vi "Module Loop.vi"(8 "error in (no error)":errorcluster, 11 "GUI Manager Module in":refnum<class "GUI Manager Module.lvclass">) -> (0 "error out":errorcluster, 3 "GUI Manager Module out":refnum<class "GUI Manager Module.lvclass">)   [LabVIEW 2020, in "VolatusGUI.lvlib" / "GUI Manager Module.lvclass"]
uses:
  GUI Manager Module.lvclass
  C:/dev/lv20CE/relink/lv-volatus/Volatus/Module/Module.lvclass
  GUI Entry.ctl
  Volatus/Module/Module.lvclass/Module.ctl
  Volatus/MessageQ/MessageQ.lvclass/MessageQ.ctl
  lv-promises/Promises/Variant/Variant.lvclass/Variant.ctl
  Volatus/Module/Module.lvclass
  Volatus/Event Reporter Identity/Event Reporter Identity.lvclass
  C:/dev/lv20CE/relink/lv-volatus/Volatus/Identity/Identity.lvclass
  Volatus/Events Summary Value/Events Summary Value.lvclass
  GUI Registration.ctl
  Volatus/MessageQ/MessageQ.lvclass
  GUI Info.ctl
  GUI Manager Module.lvclass/GUI Manager Module.ctl
  Unregister GUI.ctl
  System Status Module/System Status Module.lvclass
  VolatusConfig/VolatusConfigElement/VolatusConfigElement.lvclass
  Volatus/Roles API/Roles API.lvclass
  Visibility Data.ctl
  Position Data.ctl
  <vilib>/Utility/miscctls.llb/LVRectTypeDef.ctl
  Event Viewer Identity/Event Viewer Identity.lvclass
  Volatus/Roles API/Roles API.lvclass/Roles API.ctl
  Volatus/Module Identity/Module Identity.lvclass/Module Identity.ctl
  782c3c59-6500-4745-abed-eb8793f80122.vi
  Volatus/Module Identity/Module Identity.lvclass
  <vilib>/Utility/error.llb/Error Cluster From Error Code.vi
  lv-promises/Promises/Variant/Variant.lvclass
  lv-promises/Promises/Promise/Promise.lvclass
  VolatusGUI.lvlib
  GUIStateValue/GUIStateValue.lvclass
  Volatus/VolatusAPI/VolatusAPI.lvclass
  Volatus/Volatus.lvlib
  GUI Helper/GUI Helper.lvclass
panel:
  out "Cmd Status":cluster{"Net Color":u32, "Net Status":string}
  in  "Event Log":bool
  out "Warnings":i32
  out "Errors":i32
  in  "Role Status":T1
  in  "GUIs":T2[](array[typedef])
  # "WARN"
  # "ERR"
  # "Commands"
  # "Role"
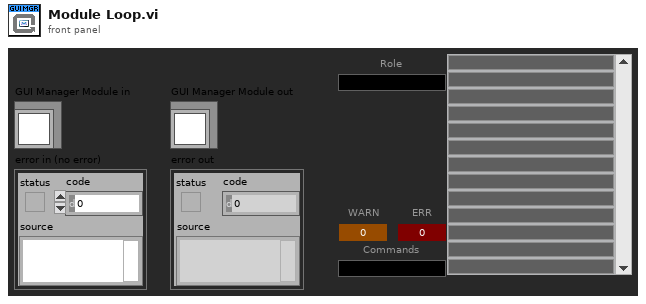
[diagram p1: front panel]
types:
  T1 = cluster{"Color":u32, "Role":string, "Select Role":bool}
  T2 = typedef "VolatusGUI.lvlib/GUI Manager Module.lvclass/GUI Entry.ctl" = cluster{"Name Color":u32, "Name":string, "Show GUI":bool, "ID":string}
  T3 = cluster{"Name Color":bool, "Name":bool, "Show GUI":bool, "ID":bool}[]
  T4 = enum32{"Invalid", "Standard", "Closed", "Hidden", "Minimized", "Maximized"}
  T5 = typedef "VolatusGUI.lvlib/GUI Registration.ctl" = cluster{"ID":string, "GUI Helper":refnum<class "MessageQ.lvclass">, "Module":refnum<class "MessageQ.lvclass">, "Info":T6, "Open":bool}
  T6 = typedef "VolatusGUI.lvlib/GUI Info.ctl" = cluster{"Color":u32, "Name":string}
  T7 = typedef "VolatusGUI.lvlib/Unregister GUI.ctl" = cluster{"Name":string}
  T8 = typedef "VolatusGUI.lvlib/Visibility Data.ctl" = cluster{"GUI ID":string, "Visible":bool}
  T9 = typedef "VolatusGUI.lvlib/Position Data.ctl" = cluster{"GUI ID":string, "Bounds":T10}
  T10 = typedef "LVRectTypeDef.ctl" = cluster{"Left":i16, "Top":i16, "Right":i16, "Bottom":i16}
  T11 = typedef "Volatus.lvlib/Events Summary.ctl" = cluster{"# Debug":i32, "# Info":i32, "# Warning":i32, "# Error":i32}
  T12 = typedef "VolatusGUI.lvlib/GUI State.ctl" = cluster{"GUI ID":string, "Visible":bool, "Visibility Set":bool, "Bounds":T10, "Bounds Set":bool}
  T13 = typedef "VolatusGUI.lvlib/GUI Manager Module.lvclass/Plugin Info.ctl" = cluster{"Path":path, "Module ID":string, "Filename":string}
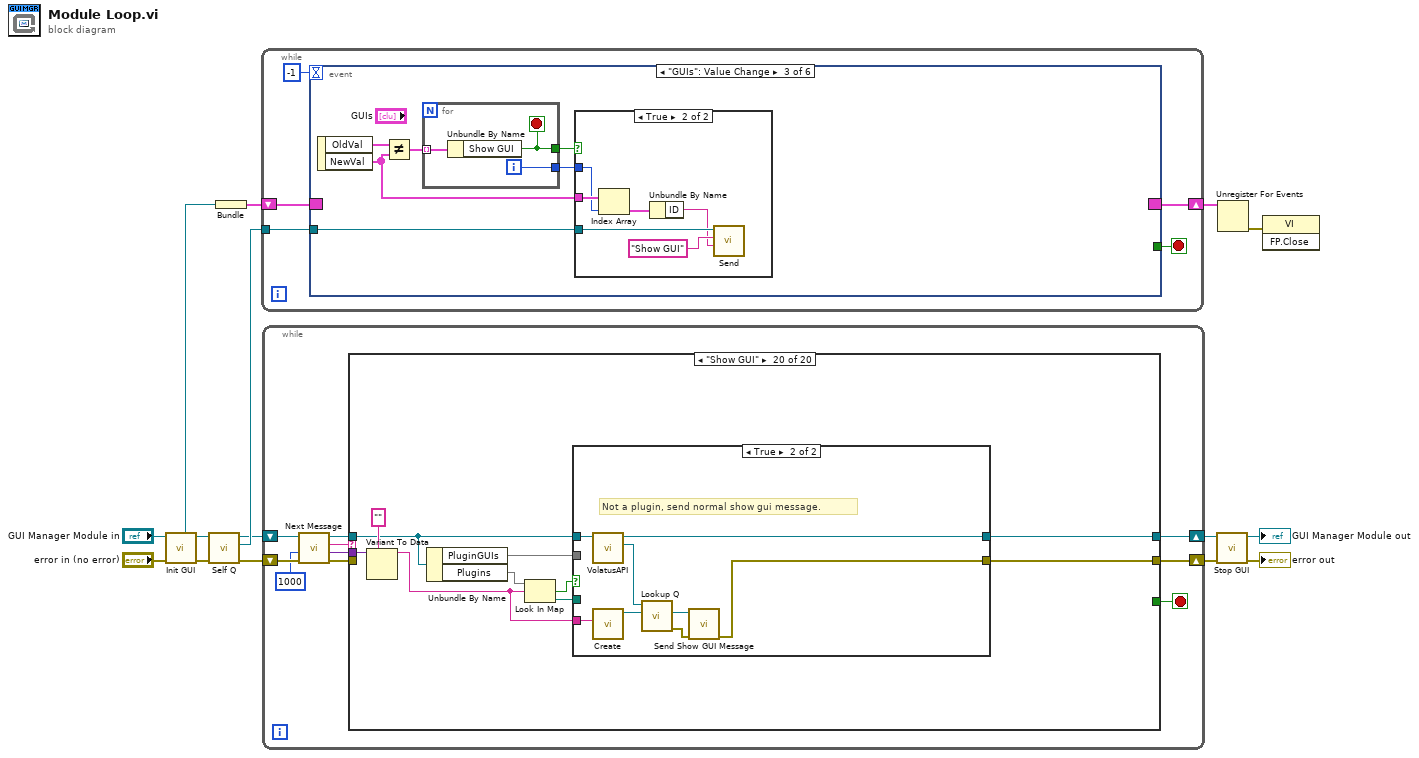
[diagram p0: block diagram]
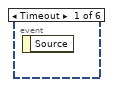
[diagram p2: hidden frame]
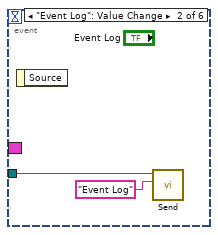
[diagram p3: hidden frame]
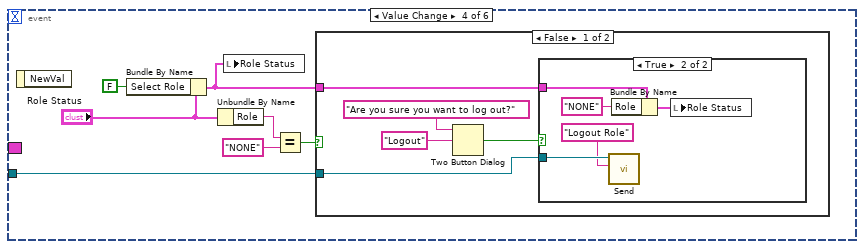
[diagram p5: hidden frame]
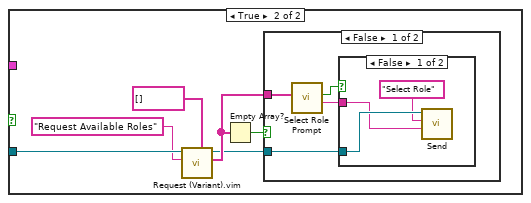
[diagram p7: hidden frame]
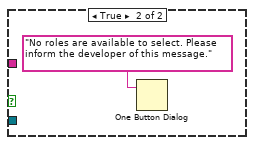
[diagram p9: hidden frame]
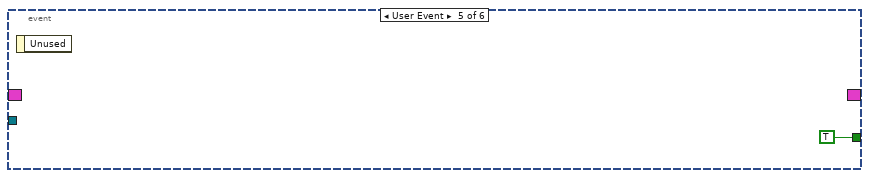
[diagram p10: hidden frame]
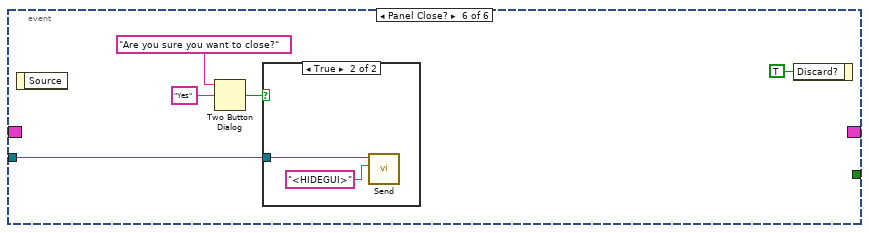
[diagram p11: hidden frame]
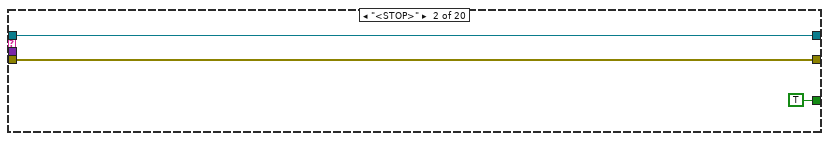
[diagram p14: hidden frame]
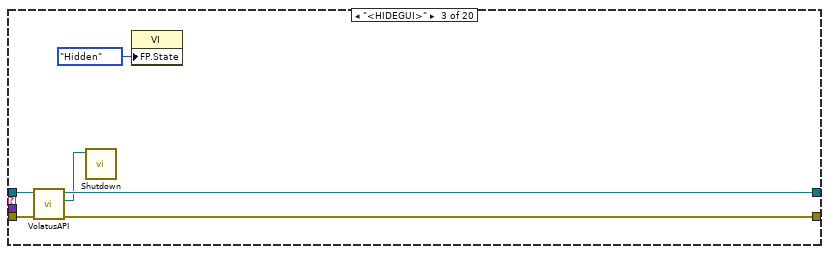
[diagram p15: hidden frame]
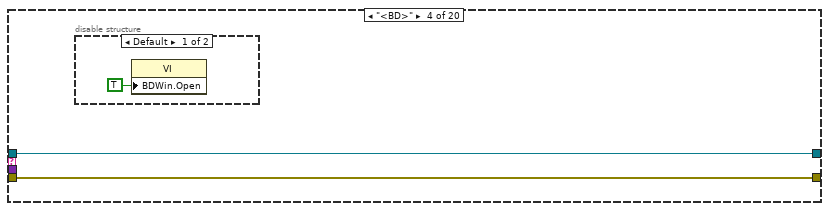
[diagram p16: hidden frame]
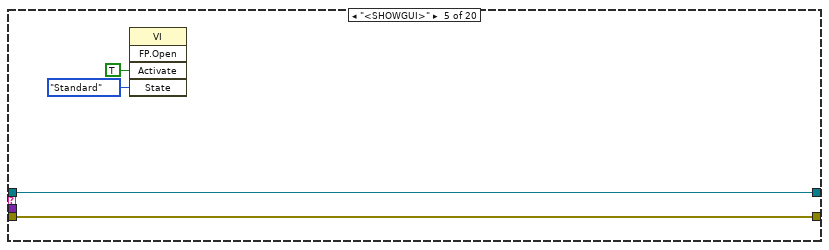
[diagram p18: hidden frame]
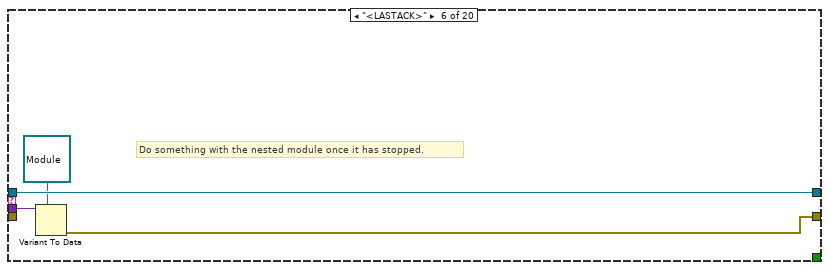
[diagram p19: hidden frame]
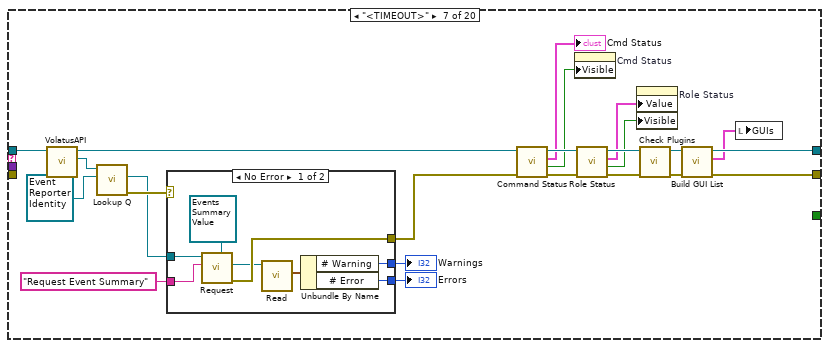
[diagram p20: hidden frame]
diagram:
  n1 = call "Init GUI.vi"("Module in"="GUI Manager Module in") -> ("Module out"=w9:refnum<class "GUI Manager Module.lvclass">, "Event Reg"=w12:refnum<event-registration>)  [unwired: 9 in]
  n2 = call "Self Q.vi"("Module in"=w9) -> ("Self Q"=w8:refnum<class "MessageQ.lvclass">, "Module out"=w7:refnum<class "GUI Manager Module.lvclass">)  [unwired: 9 in]
  n3 = Bundle("Event Reg"=w12) -> (w10:cluster{"Event Reg":refnum<event-registration>})  [unwired: 1 in]
  n4 = while {
    tunnel: w8 -> [w18]
    shift-right: [w16] -> w11
    shift-left: w10 -> [w17]
    stop <- w15 stop-if-true
    n5 = event shown="[2] \"GUIs\": Value Change" {
      selector: w17 -> [_ _ _ _ _ _]
      dyn-events: [_ _ _ _ _ _] -> w16
      timeout: -1 -> [_ _ _ _ _ _]
      tunnel: w18 -> [_ w20 w21 w42 _ w68]
      tunnel: [_ _ _ _ TRUE _] -> w15
      event Timeout {
        n6 = event-data() -> ()  [unwired: 1 in, 1 out]
      }
      event "Event Log": Value Change {
        n7 = event-data() -> ()  [unwired: 1 in, 1 out]
        n8 = call "Send.vi"("ID"="Event Log", "MessageQ in"=w20) -> ()  [unwired: 8 in, 2 out]
      }
      event "GUIs": Value Change {
        n9 = event-data() -> ("OldVal"=w26:T2[], "NewVal"=w22:T2[])  [unwired: 1 in]
        n10 = Not Equal?(x=w26, y=w22) -> (x != y?=w25:T3)
        n11 = for {
          tunnel: w25 -> [w35] mode=indexing
          tunnel: [w34] -> w24
          tunnel: [w33] -> w23
          i -> [w33]
          stop <- w34 stop-if-true
          n12 = Unbundle By Name(w35) -> ("Show GUI"=w34:bool)
        }
        n13 = case shown="True" w24 {
          tunnel: w23 -> [_ w31]
          tunnel: w22 -> [_ w32]
          tunnel: w21 -> [_ w29]
          frame False {
          }
          frame True {
            n14 = Index Array(array=w32, index=w31) -> (element=w30:T2)
            n15 = Unbundle By Name(w30) -> ("ID"=w27:string)
            n16 = call "Send.vi"("Data"=w27, "ID"="Show GUI", "MessageQ in"=w29) -> ()  [unwired: 7 in, 2 out]
          }
        }
      }
      event "Role Status.Select Role": Value Change {
        n17 = event-data() -> ()  [unwired: 1 in, 1 out]
        n18 = Bundle By Name(cluster="Role Status", "Select Role"=FALSE) -> (w36:T1)
        n19 = Unbundle By Name("Role Status") -> ("Role"=w41:string)
        n20 = local write "Role Status"(w36) -> ()
        n21 = Equal?(x=w41, y="NONE") -> (x = y?=w39:bool)
        n22 = case shown="False" w39 {
          tunnel: w42 -> [w47 w58]
          tunnel: w36 -> [w43 _]
          frame False {
            n23 = Two Button Dialog(message="Are you sure you want to log out?", 2:"Logout" ("T button name (\"OK\")")) -> (T button?=w44:bool)  [unwired: 1 in]
            n24 = case shown="True" w44 {
              tunnel: w47 -> [_ w52]
              tunnel: w43 -> [_ w50]
              frame False {
              }
              frame True {
                n25 = call "Send.vi"("ID"="Logout Role", "MessageQ in"=w52) -> ()  [unwired: 8 in, 2 out]
                n26 = Bundle By Name(cluster=w50, "Role"="NONE") -> (w48:T1)
                n27 = local write "Role Status"(w48) -> ()
              }
            }
          }
          frame True {
            n28 = call "Request (Variant).vim"("Type"=string[] [], "ID"="Request Available Roles", "MessageQ in"=w58) -> ("Value"=w54:string[], "MessageQ out"=w53:refnum<class "MessageQ.lvclass">)  [unwired: 6 in, 1 out]
            n29 = Empty Array?(array=w54) -> (empty?=w55:bool)
            n30 = case shown="False" w55 {
              tunnel: w54 -> [w62 _]
              tunnel: w53 -> [w61 _]
              frame False {
                n31 = call "Select Role Prompt.vi"("Available Roles"=w62) -> ("Selected Role"=w59:string, "Cancelled"=w60:bool)  [unwired: 9 in]
                n32 = case shown="False" w60 {
                  tunnel: w61 -> [w65 _]
                  tunnel: w59 -> [w64 _]
                  frame False {
                    n33 = call "Send.vi"("Data"=w64, "ID"="Select Role", "MessageQ in"=w65) -> ()  [unwired: 7 in, 2 out]
                  }
                  frame True {
                  }
                }
              }
              frame True {
                n34 = One Button Dialog(message="No roles are available to select. Please inform the developer of this message.") -> ()  [unwired: 1 in, 1 out]
              }
            }
          }
        }
      }
      event User Event {
        n35 = event-data() -> ()  [unwired: 1 in, 1 out]
      }
      event Panel Close? {
        n36 = event-data() -> ()  [unwired: 1 in, 1 out]
        n37 = Two Button Dialog(message="Are you sure you want to close?", 2:"Yes" ("T button name (\"OK\")")) -> (T button?=w69:bool)  [unwired: 1 in]
        n38 = case shown="True" w69 {
          tunnel: w68 -> [_ w73]
          frame False {
          }
          frame True {
            n39 = call "Send.vi"("ID"="<HIDEGUI>", "MessageQ in"=w73) -> ()  [unwired: 8 in, 2 out]
          }
        }
        n40 = event-data("Discard?"=TRUE) -> ()  [unwired: 1 in, 1 out]
      }
    }
  }
  n41 = while {
    shift-right: [w79] -> w4
    shift-left: w7 -> [w84]
    shift-right: [w78] -> w3
    shift-left: "error in (no error)" -> [w83]
    stop <- w77 stop-if-true
    n42 = call "Next Message.vi"("error in (no error)"=w83, "Timeout ms (-1)"=1000, "Module in"=w84) -> ("error out"=w82:errorcluster, "Data"=w76:variant, "ID"=w81:string, "Module out"=w80:refnum<class "GUI Manager Module.lvclass">)  [unwired: 5 in]
    n43 = case shown="\"Show GUI\"" w81 {
      tunnel: w82 -> [w85 w88 w93 w95 w100 _ _ _ _ w167 w186 _ w201 _ _ _ _ _ _ _]
      tunnel: w80 -> [w86 w89 w94 w96 w101 w105 w112 w141 w157 w165 w183 w194 w197 w215 w229 w240 w246 w251 w256 w262]
      tunnel: [w86 w89 w91 w96 w101 w105 w121 w137 w154 w164 w173 w191 w195 w212 w223 w239 w246 w251 w256 w264] -> w79
      tunnel: [w85 w88 w93 w95 w100 w102 w123 w138 w155 w166 w175 w189 w196 w209 w233 w234 w241 w247 w254 w263] -> w78
      tunnel: [_ TRUE _ _ _ _ _ _ _ _ _ _ _ _ _ _ _ _ _ _] -> w77
      tunnel: w76 -> [_ _ _ _ _ w104 _ w143 w159 _ _ w193 w202 w214 w232 _ w244 w253 _ w266]
      frame "<CLOSE>" {
      }
      frame "<STOP>" {
      }
      frame "<HIDEGUI>" {
        n44 = call "VolatusAPI.vi"("Module in"=w94) -> ("VolatusAPI"=w90:refnum<class "VolatusAPI.lvclass">, "Module out"=w91:refnum<class "GUI Manager Module.lvclass">)  [unwired: 9 in]
        n45 = call "Shutdown.vi"("VolatusAPI in"=w90) -> ()  [unwired: 9 in, 2 out]
        n46 = property class="VI"("FP.State"=T4."Hidden" ("Front Panel Window:State")) -> ()  [unwired: 2 in, 2 out]
      }
      frame "<BD>" {
        n47 = disable-structure shown="Default" {
          frame condition #0 (active) {
            n48 = property class="VI"("BDWin.Open"=TRUE ("Block Diagram Window:Open")) -> ()  [unwired: 2 in, 2 out]
          }
          frame condition #1 {
          }
        }
      }
      frame "<SHOWGUI>" {
        n49 = invoke class="VI" method="FP.Open"("Activate"=TRUE ("Activate?"), "State"=T4."Standard") -> ()  [unwired: 3 in, 5 out]
      }
      frame "<LASTACK>" {
        # "Do something with the nested module once it has stopped."
        n50 = Variant To Data(type=refnum<class "Module.lvclass"> refnum ("Volatus:Module"), Variant=w104) -> (error out=w102:errorcluster)  [unwired: 1 in, 1 out]
      }
      frame "<TIMEOUT>" {
        n51 = call "VolatusAPI.vi"("Module in"=w112) -> ("VolatusAPI"=w113:refnum<class "VolatusAPI.lvclass">, "Module out"=w110:refnum<class "GUI Manager Module.lvclass">)  [unwired: 9 in]
        n52 = call "Lookup Q.vi"("Identity"=refnum<class "Event Reporter Identity.lvclass"> refnum ("Volatus:Event Reporter Identity.lvclass"), "VolatusAPI in"=w113) -> ("error out"=w128:errorcluster, "MessageQ"=w111:refnum<class "MessageQ.lvclass">)  [unwired: 7 in, 1 out]
        n53 = case shown="No Error" w128 {
          tunnel: "Request Event Summary" ("ID") -> [w135 _]
          tunnel: [w131 _] -> w126
          tunnel: [w130 _] -> w125
          tunnel: w111 -> [w129 _]
          tunnel: [w136 _] -> w109
          frame No Error {
            n54 = call "Request.vi"("Response Type (None)"=refnum<class "Events Summary Value.lvclass"> refnum ("Volatus:Events Summary Value.lvclass"), "ID"=w135, "MessageQ in"=w129) -> ("error out"=w136:errorcluster, "Response"=w133:refnum<class "Events Summary Value.lvclass">)  [unwired: 6 in, 1 out]
            n55 = call "Read.vi"("Events Summary Value in"=w133) -> ("Events Summary"=w132:T11)  [unwired: 10 in]
            n56 = Unbundle By Name(w132) -> ("# Warning"=w131:i32, "# Error"=w130:i32)
          }
          frame Error {
          }
        }
        "Errors" <- w125
        "Warnings" <- w126
        n57 = call "Command Status.vi"("error in (no error)"=w109, "GUI Manager Module in"=w110) -> ("error out"=w108:errorcluster, "Cmd Active"=w117:bool, "Cmd Status"=→"Cmd Status":cluster{u32, string}, "GUI Manager Module out"=w119:refnum<class "GUI Manager Module.lvclass">)  [unwired: 6 in]
        n58 = property on="Cmd Status" class="Clust (strict)"("Visible"=w117) -> ()  [unwired: 2 in, 2 out]
        n59 = call "Role Status.vi"("error in (no error)"=w108, "GUI Manager Module in"=w119) -> ("error out"=w107:errorcluster, "Roles Active"=w114:bool, "Role Status"=w115:T1, "GUI Manager Module out"=w116:refnum<class "GUI Manager Module.lvclass">)  [unwired: 6 in]
        n60 = property on="Role Status" class="Clust (strict)"("Value"=w115, "Visible"=w114) -> ()  [unwired: 2 in, 2 out]
        n61 = call "Check Plugins.vi"("error in (no error)"=w107, "GUI Manager Module in"=w116) -> ("error out"=w124:errorcluster, "GUI Manager Module out"=w122:refnum<class "GUI Manager Module.lvclass">)  [unwired: 8 in]
        n62 = call "Build GUI List.vi"("error in (no error)"=w124, "GUI Manager Module in"=w122) -> ("error out"=w123:errorcluster, "GUIs"=w120:T2[], "GUI Manager Module out"=w121:refnum<class "GUI Manager Module.lvclass">)  [unwired: 7 in]
        n63 = local write "GUIs"(w120) -> ()
      }
      frame "Register GUI" {
        n64 = Variant To Data(type=T5 {"ID"="", "GUI Helper"=refnum, "Module"=refnum, "Info"={"Color"=0, "Name"=""}, "Open"=FALSE} ("GUI Registration"), Variant=w143) -> (data=w140:T5, error out=w139:errorcluster)  [unwired: 1 in]
        n65 = case shown="No Error" w139 {
          selector: w139 -> [_ w153]
          tunnel: w141 -> [w147 w152]
          tunnel: w140 -> [w145 _]
          tunnel: [_ w153] -> w138
          tunnel: [w144 w152] -> w137
          frame No Error {
            n66 = Unbundle By Name(w145) -> ("ID"=w146:string)
            n67 = in-place {
              in-place-border: w146 -> [w150]
              in-place-border: w145 -> [w149]
              n68 = in-place-cluster #1(w147) -> ("GUIs"=w151:map{string, T5})
              n69 = Insert Into Map(map in=w151, key=w150, value=w149) -> (map out=w148:map{string, T5})  [unwired: 2 out]
              n70 = in-place-cluster #1("GUIs"=w148) -> (w144:refnum<class "GUI Manager Module.lvclass">)
            }
          }
          frame Error {
          }
        }
      }
      frame "Unregister GUI" {
        n71 = Variant To Data(type=T7 {"Name"=""} ("Unregister GUI"), Variant=w159) -> (data=w156:T7, error out=w155:errorcluster)  [unwired: 1 in]
        n72 = in-place {
          in-place-border: w156 -> [w163]
          n73 = in-place-cluster #2(w157) -> ("GUIs"=w162:map{string, T5})
          n74 = Unbundle By Name(w163) -> ("Name"=w161:string)
          n75 = Remove From Map(10:w161, 11:w162) -> (3:w160:map{string, T5})  [unwired: 2 out]
          n76 = in-place-cluster #2("GUIs"=w160) -> (w154:refnum<class "GUI Manager Module.lvclass">)
        }
      }
      frame Default {
        n77 = call "Report Unhandled Message ID.vi"("error in (no error)"=w167, "Module in"=w165) -> ("error out"=w166:errorcluster, "Module out"=w164:refnum<class "GUI Manager Module.lvclass">)  [unwired: 8 in]
      }
      frame "Initialize" {
        n78 = control-ref of="This VI"() -> (w185:refnum<vi>)
        n79 = call "Send Show GUI Message.vi"("error in (no error)"=w186, "Module in"=w183) -> ("error out"=w184:errorcluster, "Module out"=w182:refnum<class "GUI Manager Module.lvclass">)  [unwired: 8 in]
        n80 = call "Launch as Nested.vi"("Register (T)"=FALSE, "error in (no error)"=w184, "GUI"=w185, "Parent in"=w182) -> ("error out"=w169:errorcluster, "Parent"=w170:refnum<class "GUI Manager Module.lvclass">)  [unwired: 5 in, 1 out]
        n81 = call "Subscribe to Roles.vi"("error in (no error)"=w169, "Module in"=w170) -> ("error out"=w187:errorcluster, "Module out"=w168:refnum<class "GUI Manager Module.lvclass">)  [unwired: 8 in]
        n82 = Unbundle By Name(w168) -> ("Title"=w177:string)
        n83 = Empty String/Path?(string/path=w177) -> (empty?=w178:bool)
        n84 = case shown="False" w178 {
          tunnel: w177 -> [w188 _]
          frame False {
            n85 = property class="VI"("Front Panel.Title"=w188) -> ()  [unwired: 2 in, 2 out]
          }
          frame True {
          }
        }
        n86 = call "Check Plugins.vi"("error in (no error)"=w187, "GUI Manager Module in"=w168) -> ("error out"=w181:errorcluster, "GUI Manager Module out"=w179:refnum<class "GUI Manager Module.lvclass">)  [unwired: 8 in]
        n87 = call "Check Plugin Visibility.vi"("error in (no error)"=w181, "GUI Manager Module in"=w179) -> ("error out"=w180:errorcluster, "GUI Manager Module out"=w174:refnum<class "GUI Manager Module.lvclass">)  [unwired: 8 in]
        n88 = call "Launch Nested.vi"("error in (no error)"=w180, "Config Element"=refnum<class "VolatusConfigElement.lvclass"> refnum, "Nested Module"=refnum<class "System Status Module.lvclass"> refnum ("VolatusGUI:System Status Module.lvclass"), "Parent in"=w174) -> ("error out"=w175:errorcluster, "Parent out"=w173:refnum<class "GUI Manager Module.lvclass">)  [unwired: 5 in, 1 out]
      }
      frame "Update Roles" {
        n89 = Variant To Data(type=refnum<class "Roles API.lvclass"> refnum ("Volatus:Roles API.lvclass"), Variant=w193) -> (data=w190:refnum<class "Roles API.lvclass">, error out=w189:errorcluster)  [unwired: 1 in]
        n90 = Bundle By Name(cluster=w194, "Roles"=w190) -> (w191:refnum<class "GUI Manager Module.lvclass">)
      }
      frame "Update Visibility" {
        n91 = Variant To Data(error in=w201, type=T8 {"GUI ID"="", "Visible"=FALSE} ("Visibility Data"), Variant=w202) -> (data=w199:T8, error out=w198:errorcluster)
        n92 = case shown="No Error" w198 {
          selector: w198 -> [_ w207]
          tunnel: w199 -> [w205 _]
          tunnel: w197 -> [w206 w208]
          tunnel: [w204 w207] -> w196
          tunnel: [w203 w208] -> w195
          frame No Error {
            n93 = call "Store Visibility.vi"("Visibility Data"=w205, "GUI Manager Module in"=w206) -> ("error out"=w204:errorcluster, "GUI Manager Module out"=w203:refnum<class "GUI Manager Module.lvclass">)  [unwired: 8 in]
          }
          frame Error {
          }
        }
      }
      frame "Update Position" {
        n94 = Variant To Data(type=T9 {"GUI ID"="", "Bounds"={"Left"=0, "Top"=0, "Right"=0, "Bottom"=0}} ("Position Message"), Variant=w214) -> (data=w211:T9, error out=w210:errorcluster)  [unwired: 1 in]
        n95 = case shown="No Error" w210 {
          selector: w210 -> [w217 w222]
          tunnel: w215 -> [w220 w221]
          tunnel: [w219 w221] -> w212
          tunnel: w211 -> [w218 _]
          tunnel: [w216 w222] -> w209
          frame No Error {
            n96 = call "Store Position.vi"("error in (no error)"=w217, "Position Message"=w218, "GUI Manager Module in"=w220) -> ("error out"=w216:errorcluster, "GUI Manager Module out"=w219:refnum<class "GUI Manager Module.lvclass">)  [unwired: 7 in]
          }
          frame Error {
          }
        }
      }
      frame "Request State" {
        n97 = call "Unpack Request.vi"("Request Data"=w232) -> ("Data"=w231:variant, "Promise"=w225:refnum<class "Promise.lvclass">)  [unwired: 8 in, 1 out]
        n98 = Variant To Data(type="", Variant=w231) -> (data=w228:string, error out=w227:errorcluster)  [unwired: 1 in]
        n99 = call "Read State.vi"("error in (no error)"=w227, "GUI ID"=w228, "GUI Manager Module in"=w229) -> ("error out"=w233:errorcluster, "GUI State"=w226:T12, "GUI Manager Module out"=w223:refnum<class "GUI Manager Module.lvclass">)  [unwired: 6 in]
        n100 = call "Create.vi"("GUI State"=w226) -> ("GUIStateValue out"=w224:refnum<class "GUIStateValue.lvclass">)  [unwired: 10 in]
        n101 = call "Resolve.vi"("error in (no error)"=w233, "Result (None)"=w224, "Promise in"=w225) -> ()  [unwired: 7 in, 2 out]
      }
      frame "Event Log" {
        n102 = call "VolatusAPI.vi"("Module in"=w240) -> ("VolatusAPI"=w238:refnum<class "VolatusAPI.lvclass">, "Module out"=w239:refnum<class "GUI Manager Module.lvclass">)  [unwired: 9 in]
        n103 = call "Lookup Q.vi"("Identity"=refnum<class "Event Viewer Identity.lvclass"> refnum ("VolatusGUI:Event Viewer Identity.lvclass"), "VolatusAPI in"=w238) -> ("error out"=w235:errorcluster, "MessageQ"=w236:refnum<class "MessageQ.lvclass">)  [unwired: 7 in, 1 out]
        n104 = call "Send Show GUI Message.vi"("error in (no error)"=w235, "MessageQ"=w236) -> ("error out"=w234:errorcluster)  [unwired: 9 in]
      }
      frame "Request Available Roles" {
        n105 = call "Unpack Request.vi"("Request Data"=w244) -> ("Promise"=w243:refnum<class "Promise.lvclass">)  [unwired: 8 in, 2 out]
        n106 = Unbundle By Name(w246) -> ("Roles"=w245:refnum<class "Roles API.lvclass">)
        n107 = call "Available Roles.vi"("Roles API in"=w245) -> ("Roles Available"=w242:string[])  [unwired: 8 in, 2 out]
        n108 = call "Resolve Variant.vi"("Value"=w242, "Promise in"=w243) -> ("error out"=w241:errorcluster)  [unwired: 8 in, 1 out]
      }
      frame "Select Role" {
        n109 = Variant To Data(type="", Variant=w253) -> (data=w249:string, error out=w248:errorcluster)  [unwired: 1 in]
        n110 = Unbundle By Name(w251) -> ("Roles"=w250:refnum<class "Roles API.lvclass">)
        n111 = call "Select Role.vi"("error in (no error)"=w248, "Select Role"=w249, "Roles API in"=w250) -> ("error out"=w247:errorcluster)  [unwired: 7 in, 1 out]
      }
      frame "Logout Role" {
        n112 = Unbundle By Name(w256) -> ("Roles"=w255:refnum<class "Roles API.lvclass">)
        n113 = call "Logout Role.vi"("Roles API in"=w255) -> ("error out"=w254:errorcluster)  [unwired: 9 in, 1 out]
      }
      frame "Show GUI" {
        n114 = Variant To Data(type="", Variant=w266) -> (data=w257:string)  [unwired: 1 in, 1 out]
        n115 = Unbundle By Name(w262) -> ("PluginGUIs"=w258:map{path, T13}, "Plugins"=w261:map{string, path})
        n116 = Look In Map(map=w261, key=w257) -> (key not found?=w260:bool, value=w259:path)  [unwired: 1 in]
        n117 = case shown="True" w260 {
          tunnel: [w270 w316] -> w264
          tunnel: [w271 w311] -> w263
          tunnel: w262 -> [w275 w310]
          tunnel: w259 -> [w267 _]
          tunnel: w258 -> [w276 _]
          tunnel: w257 -> [w268 w309]
          frame False {
            n118 = call "VolatusAPI.vi"("Module in"=w275) -> ("VolatusAPI"=w273:refnum<class "VolatusAPI.lvclass">, "Module out"=w269:refnum<class "GUI Manager Module.lvclass">)  [unwired: 9 in]
            n119 = Look In Map(map=w276, key=w267) -> (key not found?=w272:bool, value=w274:T13)  [unwired: 1 in]
            n120 = case shown="False" w272 {
              tunnel: w274 -> [w277 _]
              tunnel: w273 -> [w282 w293]
              tunnel: [w280 w295] -> w271
              tunnel: [w279 w294] -> w270
              tunnel: w269 -> [w278 w298]
              tunnel: w268 -> [_ w297]
              tunnel: w267 -> [_ w296]
              frame False {
                # "Configured PluginGUI"
                n121 = Unbundle By Name(w277) -> ("Module ID"=w281:string)
                n122 = call "Create.vi"("ID"=w281) -> ("Module Identity out"=w285:refnum<class "Module Identity.lvclass">)  [unwired: 10 in]
                n123 = call "Lookup Q.vi"("Identity"=w285, "VolatusAPI in"=w282) -> ("error out"=w283:errorcluster, "MessageQ"=w284:refnum<class "MessageQ.lvclass">)  [unwired: 7 in, 1 out]
                n124 = case shown="No Error" w283 {
                  tunnel: w284 -> [w288 _]
                  tunnel: [w287 w289] -> w280
                  tunnel: [w286 w290] -> w279
                  tunnel: w278 -> [w286 w292]
                  tunnel: w277 -> [_ w291]
                  frame No Error {
                    n125 = call "Send Show GUI Message.vi"("MessageQ"=w288) -> ("error out"=w287:errorcluster)  [unwired: 10 in]
                  }
                  frame Error {
                    n126 = call "Launch Plugin (Info).vi"("Plugin Info"=w291, "GUI Manager Module in"=w292) -> ("error out"=w289:errorcluster, "GUI Manager Module out"=w290:refnum<class "GUI Manager Module.lvclass">)  [unwired: 8 in]
                  }
                }
              }
              frame True {
                # "Unconfigured Plugin"
                n127 = call "Create.vi"("ID"=w297) -> ("Module Identity out"=w301:refnum<class "Module Identity.lvclass">)  [unwired: 10 in]
                n128 = call "Lookup Q.vi"("Identity"=w301, "VolatusAPI in"=w293) -> ("error out"=w299:errorcluster, "MessageQ"=w300:refnum<class "MessageQ.lvclass">)  [unwired: 7 in, 1 out]
                n129 = case shown="Error .." w299 {
                  tunnel: w300 -> [w304 _]
                  tunnel: [w303 w305] -> w295
                  tunnel: [w302 w306] -> w294
                  tunnel: w298 -> [w302 w308]
                  tunnel: w296 -> [_ w307]
                  frame No Error {
                    n130 = call "Send Show GUI Message.vi"("MessageQ"=w304) -> ("error out"=w303:errorcluster)  [unwired: 10 in]
                  }
                  frame Error {
                    n131 = call "Launch Plugin (Path).vi"("Path"=w307, "GUI Manager Module in"=w308) -> ("error out"=w305:errorcluster, "GUI Manager Module out"=w306:refnum<class "GUI Manager Module.lvclass">)  [unwired: 8 in]
                  }
                }
              }
            }
          }
          frame True {
            # "Not a plugin, send normal show gui message."
            n132 = call "VolatusAPI.vi"("Module in"=w310) -> ("VolatusAPI"=w315:refnum<class "VolatusAPI.lvclass">, "Module out"=w316:refnum<class "GUI Manager Module.lvclass">)  [unwired: 9 in]
            n133 = call "Create.vi"("ID"=w309) -> ("Module Identity out"=w314:refnum<class "Module Identity.lvclass">)  [unwired: 10 in]
            n134 = call "Lookup Q.vi"("Identity"=w314, "VolatusAPI in"=w315) -> ("error out"=w312:errorcluster, "MessageQ"=w313:refnum<class "MessageQ.lvclass">)  [unwired: 7 in, 1 out]
            n135 = call "Send Show GUI Message.vi"("error in (no error)"=w312, "MessageQ"=w313) -> ("error out"=w311:errorcluster)  [unwired: 9 in]
          }
        }
      }
    }
  }
  n136 = call "Stop GUI.vi"("error in (no error)"=w3, "Module in"=w4) -> ("error out"=→"error out":errorcluster, "Module out"=→"GUI Manager Module out":refnum<class "GUI Manager Module.lvclass">)  [unwired: 8 in]
  n137 = Unregister For Events(event registration refnum=w11) -> (error out=w13:errorcluster)  [unwired: 1 in]
  n138 = invoke class="VI" method="FP.Close"(error in=w13) -> ()  [unwired: 2 in, 3 out]
